vi "Sound_Mix.vi"(0 "Sounds":i32, 1 "Priority":i32=99, 2 "Music on":bool, 3 "Music Position":i32, 5 "Bank":cluster{"Y":dbl[]}[](array[cluster]), 7 "Current":dbl[](array[numeric]), 9 "Position":i32, 11 "error in":errorcluster) -> (4 "Block":dbl[](array[numeric]), 6 "Current out":dbl[](array[numeric]), 8 "Position out":i32, 10 "Priority out":i32, 13 "Music Position out":i32, 15 "error out":errorcluster)   [LabVIEW 2020, in "GH_Audio.lvlib"]
doc: "One audio block (512 samples): picks the most important effect of the sound bits; it replaces the running effect when that one has ended or is not more important. Returns the next samples of the running effect, filled with silence, plus the music (bank entry 13, volume 0.3) from Music Position, looping seamlessly."
uses:
  GH_Audio.lvlib
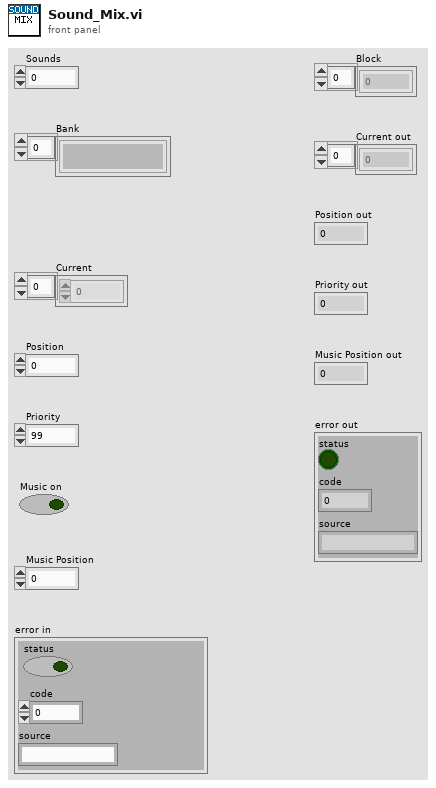
[diagram p1: front panel]
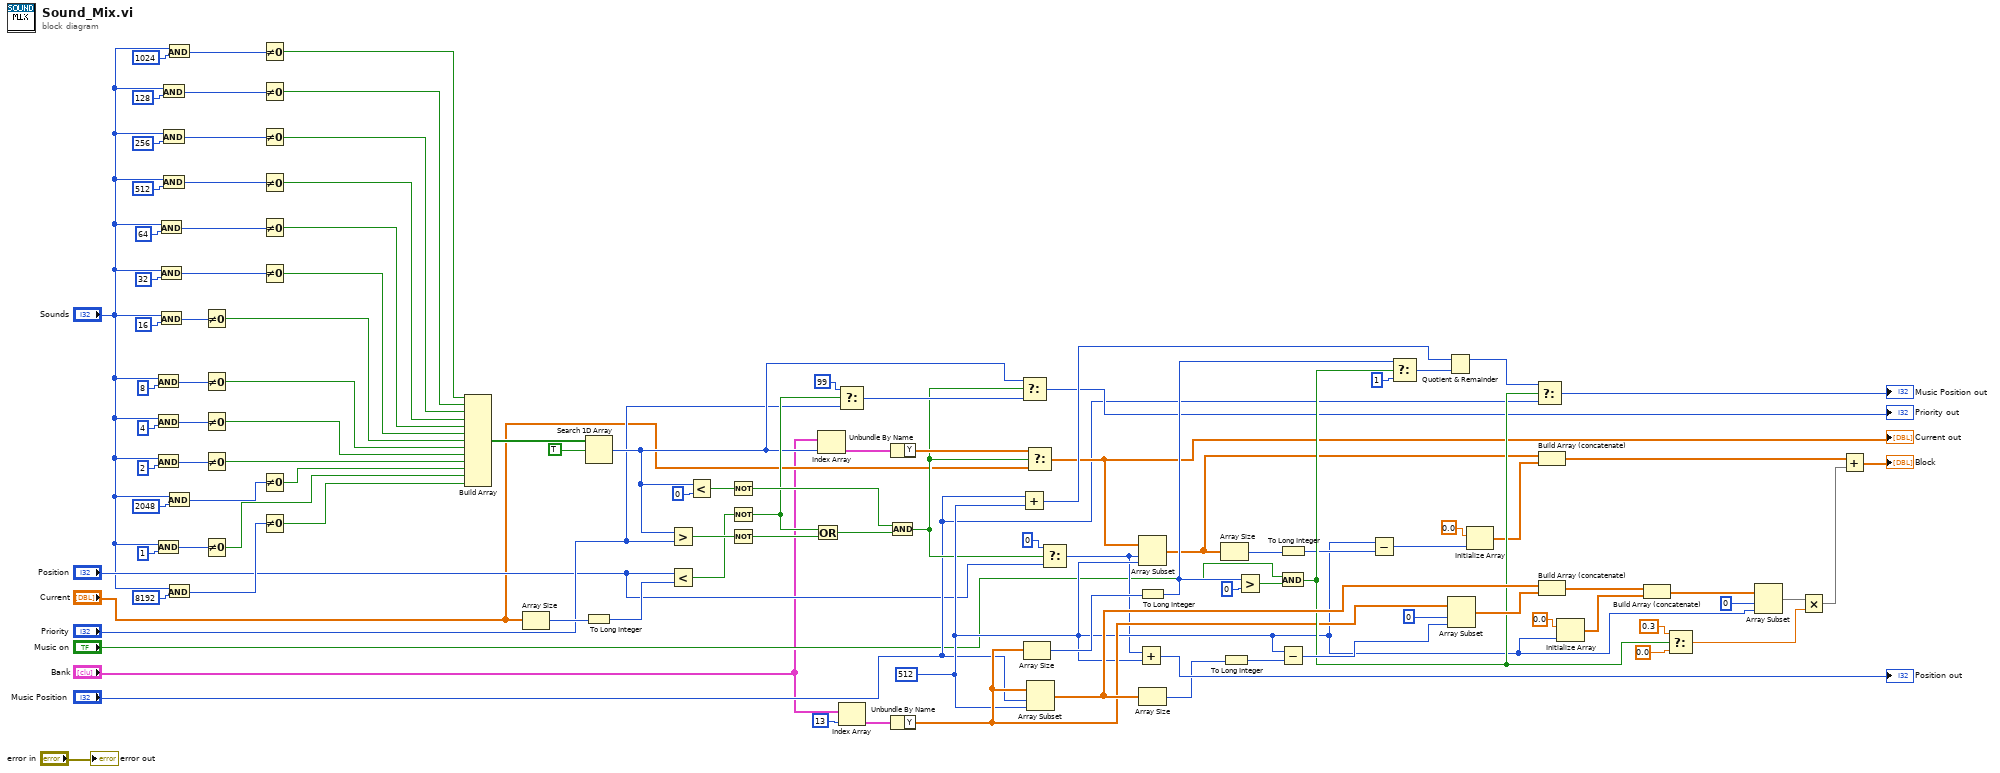
[diagram p0: block diagram]
diagram:
  w70 = 512
  n1 = And(x="Sounds", y=8) -> (x .and. y?=w31:i32)
  n2 = And(x="Sounds", y=4) -> (x .and. y?=w34:i32)
  n3 = And(x="Sounds", y=2) -> (x .and. y?=w37:i32)
  n4 = And(x="Sounds", y=1) -> (x .and. y?=w43:i32)
  n5 = And(x="Sounds", y=64) -> (x .and. y?=w22:i32)
  n6 = And(x="Sounds", y=32) -> (x .and. y?=w25:i32)
  n7 = And(x="Sounds", y=16) -> (x .and. y?=w28:i32)
  n8 = And(x="Sounds", y=128) -> (x .and. y?=w13:i32)
  n9 = And(x="Sounds", y=256) -> (x .and. y?=w16:i32)
  n10 = And(x="Sounds", y=512) -> (x .and. y?=w19:i32)
  n11 = And(x="Sounds", y=1024) -> (x .and. y?=w10:i32)
  n12 = And(x="Sounds", y=2048) -> (x .and. y?=w40:i32)
  n13 = And(x="Sounds", y=8192) -> (x .and. y?=w46:i32)
  n14 = Not Equal To 0?(x=w28) -> (x != 0?=w29:bool)
  n15 = Not Equal To 0?(x=w31) -> (x != 0?=w32:bool)
  n16 = Not Equal To 0?(x=w34) -> (x != 0?=w35:bool)
  n17 = Not Equal To 0?(x=w37) -> (x != 0?=w38:bool)
  n18 = Not Equal To 0?(x=w43) -> (x != 0?=w44:bool)
  n19 = Not Equal To 0?(x=w10) -> (x != 0?=w11:bool)
  n20 = Not Equal To 0?(x=w13) -> (x != 0?=w14:bool)
  n21 = Not Equal To 0?(x=w16) -> (x != 0?=w17:bool)
  n22 = Not Equal To 0?(x=w19) -> (x != 0?=w20:bool)
  n23 = Not Equal To 0?(x=w22) -> (x != 0?=w23:bool)
  n24 = Not Equal To 0?(x=w25) -> (x != 0?=w26:bool)
  n25 = Not Equal To 0?(x=w40) -> (x != 0?=w41:bool)
  n26 = Not Equal To 0?(x=w46) -> (x != 0?=w47:bool)
  n27 = Build Array(w11, w14, w17, w20, w23, w26, w29, w32, w35, w38, w41, w44, w47) -> (w48:bool[])
  n28 = Array Size(array="Current") -> (size(s)=w51:i32)
  n29 = To Long Integer(number=w51) -> (32bit integer=w52:i32)
  n30 = Search 1D Array(1D array=w48, element=TRUE) -> (index of element=w50:i32)  [unwired: 1 in]
  n31 = Greater?(x=w50, y="Priority") -> (0:w58:bool)
  n32 = Less?(x="Position", y=w52) -> (x < y?=w53:bool)
  n33 = Less?(x=w50, y=0) -> (x < y?=w56:bool)
  n34 = Not(x=w56) -> (.not. x?=w57:bool)
  n35 = Not(x=w53) -> (.not. x?=w54:bool)
  n36 = Not(x=w58) -> (.not. x?=w59:bool)
  n37 = Or(x=w54, y=w59) -> (x .or. y?=w60:bool)
  n38 = Index Array(array="Bank", index=w50) -> (element=w62:cluster{"Y":dbl[]})
  n39 = Select(t=99, s=w54, f="Priority") -> (s? t:f=w68:i32)
  n40 = Index Array(array="Bank", index=13) -> (element=w79:cluster{"Y":dbl[]})
  n41 = And(x=w57, y=w60) -> (x .and. y?=w61:bool)
  n42 = Unbundle By Name(w62) -> ("Y"=w63:dbl[])
  n43 = Unbundle By Name(w79) -> ("Y"=w80:dbl[])
  n44 = Select(t=w50, s=w61, f=w68) -> (s? t:f=→"Priority out":i32)
  n45 = Add(x="Music Position", y=w70) -> (x+y=w103:i32)
  n46 = Array Size(array=w80) -> (size(s)=w81:i32)
  n47 = Select(t=w63, s=w61, f="Current") -> (s? t:f=w64:dbl[])
  "Current out" <- w64
  n48 = Array Subset(array=w80, index="Music Position", length=w70) -> (w86:dbl[])
  n49 = Select(t=0, s=w61, f="Position") -> (s? t:f=w66:i32)
  n50 = Add(x=w66, y=w70) -> (x+y=→"Position out":i32)
  n51 = Array Subset(array=w64, index=w66, length=w70) -> (w71:dbl[])
  n52 = To Long Integer(number=w81) -> (32bit integer=w82:i32)
  n53 = Array Size(array=w86) -> (size(s)=w88:i32)
  n54 = Array Size(array=w71) -> (size(s)=w73:i32)
  n55 = To Long Integer(number=w88) -> (32bit integer=w89:i32)
  n56 = Greater?(x=w82, y=0) -> (0:w84:bool)
  n57 = To Long Integer(number=w73) -> (32bit integer=w74:i32)
  n58 = And(x="Music on", y=w84) -> (x .and. y?=w85:bool)
  n59 = Subtract(x=w70, y=w89) -> (x-y=w90:i32)
  n60 = Subtract(x=w70, y=w74) -> (x-y=w75:i32)
  n61 = Select(t=w82, s=w85, f=1) -> (s? t:f=w105:i32)
  n62 = Quotient & Remainder(x=w103, y=w105) -> (x-y*floor(x/y)=w106:i32)  [unwired: 1 out]
  n63 = Array Subset(array=w80, index=0, length=w90) -> (w91:dbl[])
  n64 = Initialize Array(0.0, w75) -> (w76:dbl[])
  n65 = Select(t=w106, s=w85, f="Music Position") -> (s? t:f=→"Music Position out":i32)
  n66 = Build Array (concatenate)(w71, w76) -> (w77:dbl[])
  n67 = Build Array (concatenate)(w86, w91) -> (w92:dbl[])
  n68 = Initialize Array(0.0, w70) -> (w94:dbl[])
  n69 = Build Array (concatenate)(w92, w94) -> (w95:dbl[])
  n70 = Select(t=0.3, s=w85, f=0.0) -> (s? t:f=w100:dbl)
  n71 = Array Subset(array=w95, index=0, length=w70) -> (w97:dbl[])
  n72 = Multiply(x=w97, y=w100) -> (x*y=w101:dbl[])
  n73 = Add(x=w77, y=w101) -> (x+y=→"Block":dbl[])
  "error out" <- "error in"
